vi "Connect.vi"(8 "error in (no error)":errorcluster, 11 "ImageHandler:DT-ImageHandler in":refnum<class "DT-ImageHandler.lvclass">) -> (0 "error out":errorcluster, 1 "Serial Number":string, 2 "Sensor Status":i32, 3 "ImageHandler:DT-ImageHandler out":refnum<class "DT-ImageHandler.lvclass">)   [LabVIEW 2022 SP3, in "ImageHandler.lvlib" / "DT-ImageHandler.lvclass"]
uses:
  DT-ImageHandler.lvclass
  C:/Program Files/National Instruments/LabVIEW 2025/vi.lib/ActorFramework/Actor/Actor.lvclass
  <vilib>/ActorFramework/Actor/Actor.lvclass/Actor.ctl
  ImageHandler - Controller -- Interface/ImageHandler - Controller -- Interface Messages/Log Message Msg/Log Message Msg.lvclass/Log Message Msg.ctl
  <vilib>/ActorFramework/Message Enqueuer/Message Enqueuer.lvclass/Message Enqueuer.ctl
  ImageHandler - Controller -- Interface/ImageHandler - Controller -- Interface Messages/Log Message Msg/Log Message Msg.lvclass
  C:/Program Files/National Instruments/LabVIEW 2025/vi.lib/ActorFramework/Message/Message.lvclass
  DT-ImageHandler.lvclass/DT-ImageHandler.ctl
  <vilib>/ActorFramework/Actor/Actor.lvclass
  xPanelWrapperLvLib/xPanelWrapper.lvlib
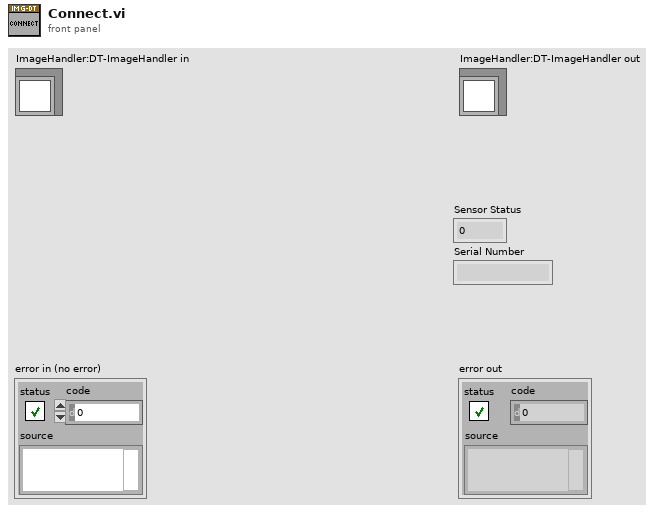
[diagram p1: front panel]
types:
  T1 = typedef "Paths.ctl" = cluster{"Configuration":path, "Event Logs":path, "Error Logs":path, "Calibration":path, "Settings.ini":path, "UserInfo.bin":path, "TimeStamp File":path, "FileCounter.txt":path}
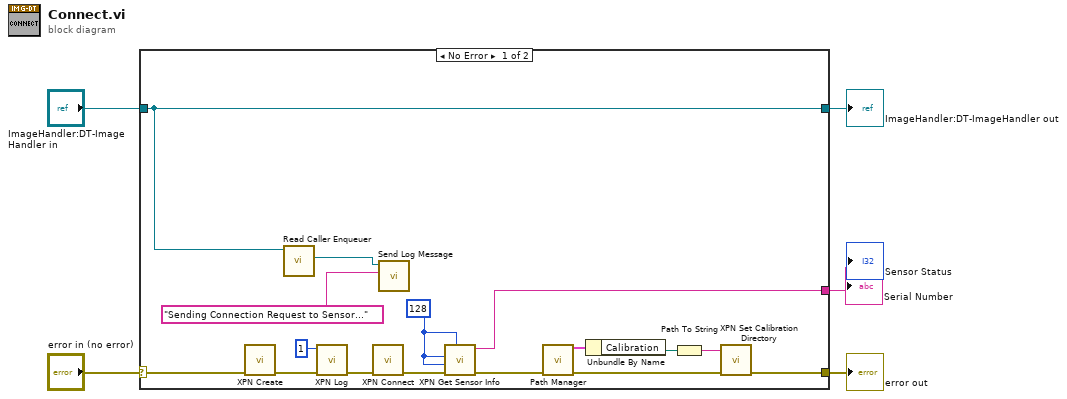
[diagram p0: block diagram]
diagram:
  n1 = case shown="No Error" "error in (no error)" {
    selector: "error in (no error)" -> [w21 w23]
    tunnel: [w11 w23] -> w4
    tunnel: [w10 w22] -> w2
    tunnel: "ImageHandler:DT-ImageHandler in" -> [w10 w22]
    tunnel: [w15 _] -> w1
    frame No Error {
      w12 = 128
      n2 = call "XPN Create.vi"("error in (no error)"=w21) -> ("error out"=w18:errorcluster)  [unwired: 9 in, 1 out]
      n3 = call <vilib>:"Read Caller Enqueuer.vi"("Actor"=w10) -> ("Caller Enqueuer"=w20:refnum<class "Message Enqueuer.lvclass">)  [unwired: 10 in]
      n4 = call "XPN Log.vi"("error in (no error)"=w18, "enable"=1) -> ("error out"=w14:errorcluster)  [unwired: 8 in, 1 out]
      n5 = call "XPN Connect.vi"("error in (no error)"=w14) -> ("error out"=w17:errorcluster)  [unwired: 9 in, 1 out]
      n6 = call "Send Log Message.vi"("Log Message"="Sending Connection Request to Sensor...", "Message Enqueuer"=w20) -> ()  [unwired: 8 in, 2 out]
      n7 = call "XPN Get Sensor Info.vi"("height"=w12, "error in (no error)"=w17, "width"=w12, "snSize"=w12) -> ("error out"=w16:errorcluster, "serialNumber out"=w15:string)  [unwired: 3 in, 3 out]
      n8 = call "Path Manager.vi"("error in (no error)"=w16) -> ("Cluster"=w8:T1, "Error out"=w9:errorcluster)  [unwired: 13 in]
      n9 = Unbundle By Name(w8) -> ("Calibration"=w6:path)
      n10 = Path To String(path=w6) -> (string=w7:string)
      n11 = call "XPN Set Calibration Directory.vi"("error in (no error)"=w9, "dirPath"=w7) -> ("error out"=w11:errorcluster)  [unwired: 8 in, 1 out]
    }
    frame Error {
    }
  }
  "error out" <- w4
  "ImageHandler:DT-ImageHandler out" <- w2
  "Serial Number" <- w1
